vi "Process Test Procedure.vi"(10 "Test Procedure File Name":string, 11 "Manual Tests Folder":path=path "C:/Users/Public/Documents/svelderrainruiz/Manual Tests") -> (3 "TestProcedure":T1)   [LabVIEW 2026, in "testCoordinator.lvlib"]
uses:
  testCoordinator.lvlib
  Test Procedure.ctl
panel:
  out "Setup Note":string
  out "Cleanup":string
  out "Main":string
  out "Setup":string
  out "Scope":string
  out "String":string
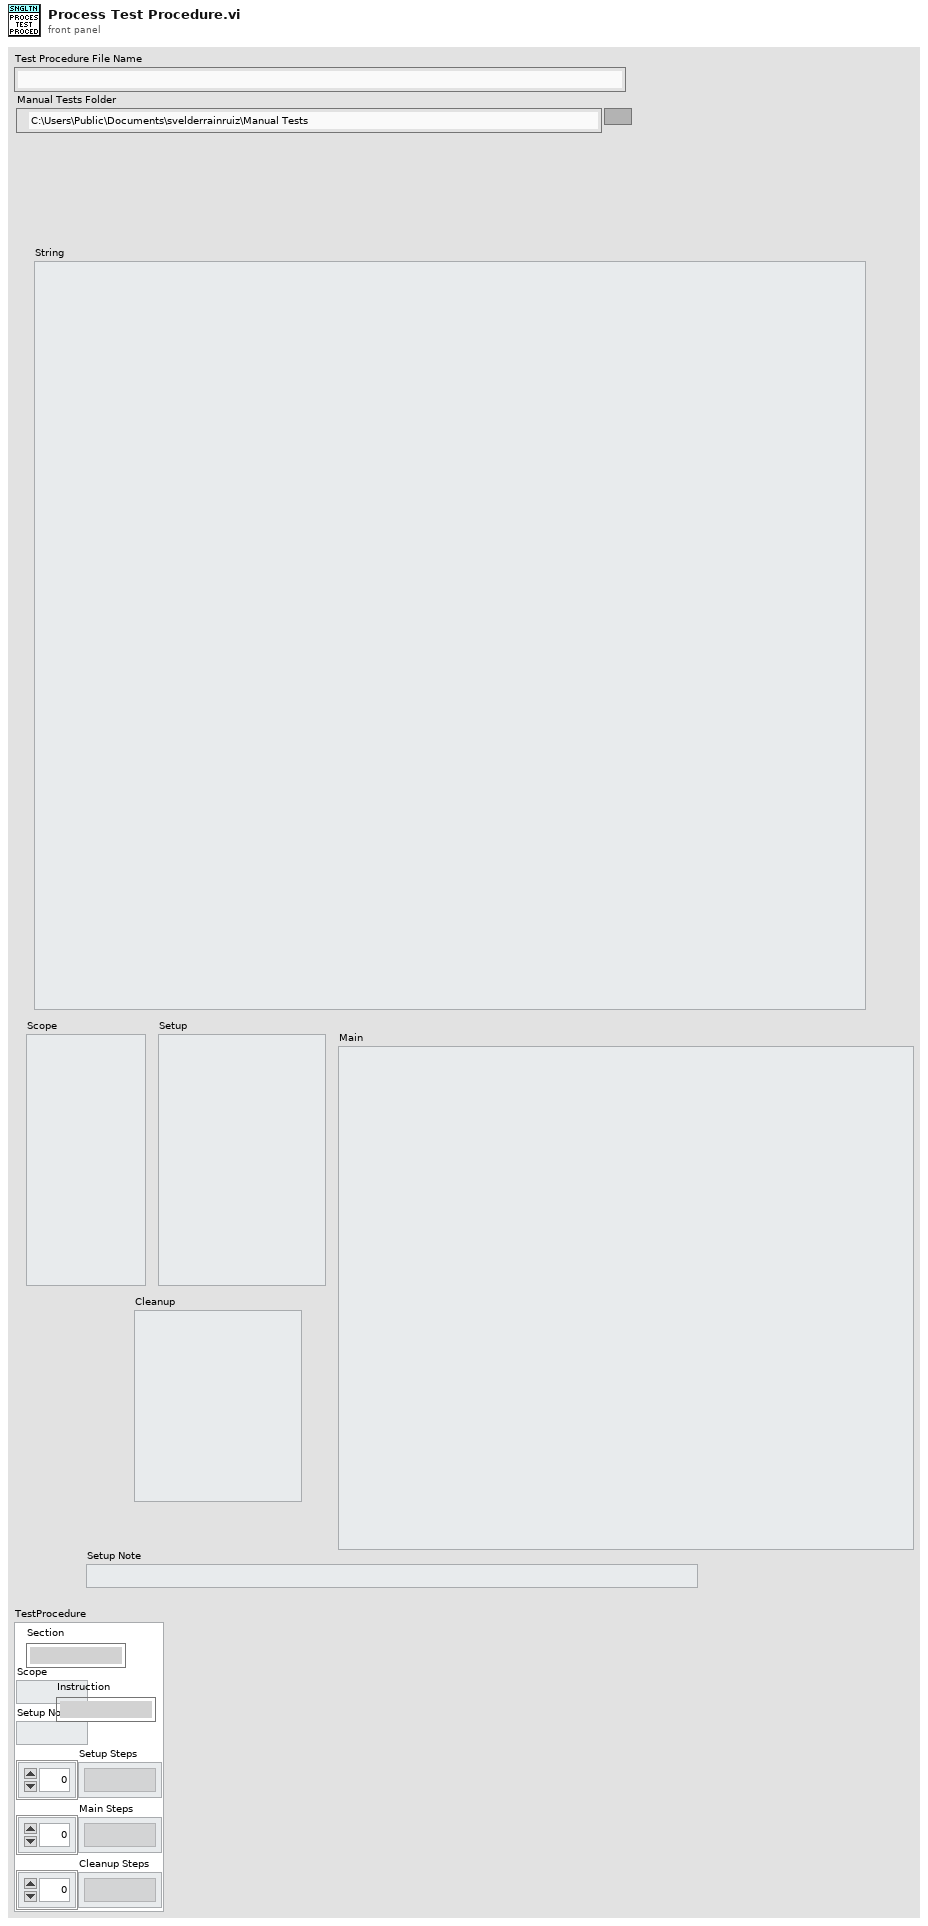
[diagram p1: front panel]
types:
  T1 = typedef "Test Procedure.ctl" = cluster{"Scope":string, "Setup Note":string, "Setup Steps":string[], "Main Steps":string[], "Cleanup Steps":string[], "Section":string, "Instruction":string}
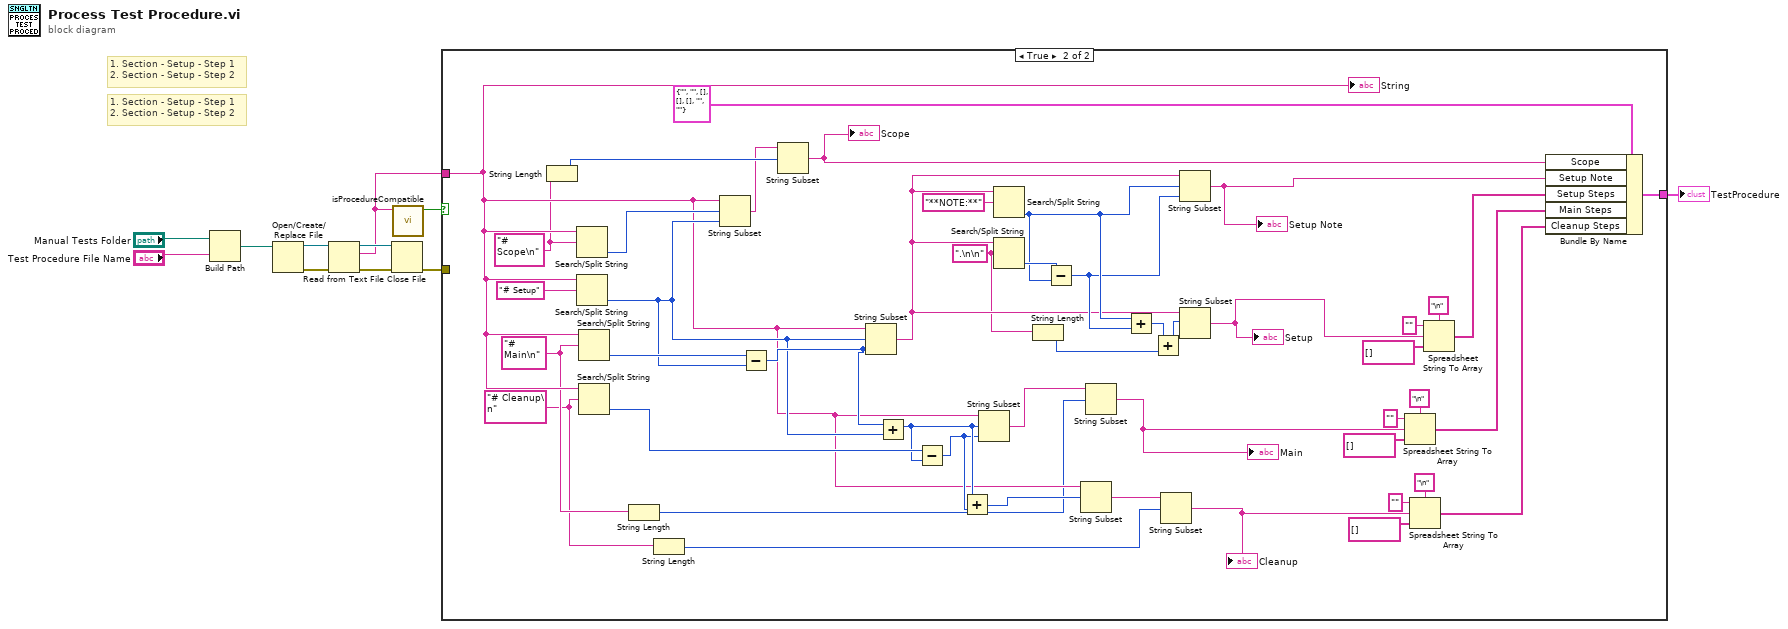
[diagram p0: block diagram]
diagram:
  # "1. Section - Setup - Step 1\n2. Section - Setup - Step 2"
  # "1. Section - Setup - Step 1\n2. Section - Setup - Step 2"
  n1 = Build Path(base path="Manual Tests Folder", name or relative path="Test Procedure File Name") -> (appended path=w5:path)
  n2 = Open/Create/Replace File(file path (use dialog)=w5) -> (refnum out=w6:refnum<file>, error out=w9:errorcluster)  [unwired: 5 in, 1 out]
  n3 = Read from Text File(file (use dialog)=w6, error in=w9) -> (refnum out=w7:refnum<file>, text=w2:string, error out=w8:errorcluster)  [unwired: 2 in, 1 out]
  n4 = Close File(refnum=w7, error in=w8) -> (error out=w3:errorcluster)  [unwired: 1 out]
  n5 = call "isProcedureCompatible.vi"("Manual Test Data"=w2) -> ("Compatible"=w4:bool)  [unwired: 10 in]
  n6 = case shown="True" w4 {
    tunnel: w3 -> [_ _]
    tunnel: w2 -> [_ w38]
    tunnel: [_ w12] -> w1
    frame False {
    }
    frame True {
      w42 = ".\n\n" ("search string/char (-)")
      w29 = "# Cleanup\n" ("search string/char (-)")
      w33 = "# Main\n" ("search string/char (-)")
      w37 = "# Scope\n" ("search string/char (-)")
      n7 = String Length(string=w37) -> (length=w36:i32)
      n8 = Search/Split String(string=w38, search string/char (-)=w37) -> (offset of match=w57:i32)  [unwired: 1 in, 2 out]
      n9 = Search/Split String(string=w38, search string/char (-)="# Setup") -> (offset of match=w54:i32)  [unwired: 1 in, 2 out]
      n10 = Search/Split String(string=w38, search string/char (-)=w33) -> (offset of match=w56:i32)  [unwired: 1 in, 2 out]
      n11 = Search/Split String(string=w38, search string/char (-)=w29) -> (offset of match=w53:i32)  [unwired: 1 in, 2 out]
      n12 = String Length(string=w33) -> (length=w31:i32)
      n13 = String Length(string=w29) -> (length=w28:i32)
      n14 = String Subset(string=w38, offset (0)=w57, length (rest)=w54) -> (substring=w35:string)
      n15 = Subtract(x=w56, y=w54) -> (x-y=w55:i32)
      n16 = String Subset(string=w35, offset (0)=w36) -> (substring=w34:string)  [unwired: 1 in]
      "Scope" <- w34
      n17 = String Subset(string=w38, offset (0)=w54, length (rest)=w55) -> (substring=w43:string)
      n18 = Add(x=w55, y=w54) -> (x+y=w52:i32)
      n19 = Subtract(x=w53, y=w52) -> (x-y=w51:i32)
      n20 = Add(x=w52, y=w51) -> (x+y=w50:i32)
      n21 = String Subset(string=w38, offset (0)=w52, length (rest)=w51) -> (substring=w32:string)
      n22 = Search/Split String(string=w43, search string/char (-)="**NOTE:**") -> (offset of match=w45:i32)  [unwired: 1 in, 2 out]
      n23 = Search/Split String(string=w43, search string/char (-)=w42) -> (offset of match=w47:i32)  [unwired: 1 in, 2 out]
      n24 = String Length(string=w42) -> (length=w40:i32)
      n25 = Subtract(x=w47, y=w45) -> (x-y=w44:i32)
      n26 = String Subset(string=w38, offset (0)=w50) -> (substring=w30:string)  [unwired: 1 in]
      n27 = String Subset(string=w32, offset (0)=w31) -> (substring=w19:string)  [unwired: 1 in]
      "Main" <- w19
      n28 = Add(x=w45, y=w44) -> (x+y=w41:i32)
      n29 = Add(x=w41, y=w40) -> (x+y=w39:i32)
      n30 = String Subset(string=w30, offset (0)=w28) -> (substring=w14:string)  [unwired: 1 in]
      "Cleanup" <- w14
      n31 = String Subset(string=w43, offset (0)=w45, length (rest)=w44) -> (substring=w46:string)
      "Setup Note" <- w46
      n32 = String Subset(string=w43, offset (0)=w39) -> (substring=w24:string)  [unwired: 1 in]
      "Setup" <- w24
      n33 = Spreadsheet String To Array(delimiter (Tab)="\n", format string="", spreadsheet string=w19, array type (2D Dbl)=string[] [] ("substring")) -> (array=w18:string[])
      n34 = Spreadsheet String To Array(delimiter (Tab)="\n", format string="", spreadsheet string=w14, array type (2D Dbl)=string[] [] ("substring")) -> (array=w13:string[])
      n35 = Spreadsheet String To Array(delimiter (Tab)="\n", format string="", spreadsheet string=w24, array type (2D Dbl)=string[] [] ("substring")) -> (array=w23:string[])
      n36 = Bundle By Name(cluster=T1 {"Scope"="", "Setup Note"="", "Setup Steps"=[], "Main Steps"=[], "Cleanup Steps"=[], "Section"="", "Instruction"=""}, "Scope"=w34, "Setup Note"=w46, "Setup Steps"=w23, "Main Steps"=w18, "Cleanup Steps"=w13) -> (w12:T1)
      "String" <- w38
    }
  }
  "TestProcedure" <- w1
